vi "Get Default Value.vi"(8 "error in":errorcluster, 9 "project refnum":refnum<vi>, 10 "measurement_signature":T2, 11 "gRPCid in":T1) -> (0 "error out":errorcluster, 3 "default value":variant)   [LabVIEW 2021, in "NI Measurement V2 Client Generator Runtime.lvlib"]
uses:
  NI Measurement V2 Client Generator Runtime.lvlib
  <vilib>/gRPC/Generated APIs/ni/measurementlink/measurement/v2/Measurement Service Client V2/RPC Messages/ni_measurementlink_measurement_v2_MeasurementSignature.ctl
  <vilib>/gRPC/Generated APIs/ni/measurementlink/measurement/v2/Measurement Service Client V2/RPC Messages/ni_measurementlink_measurement_v2_ConfigurationParameter.ctl
  <vilib>/gRPC/Generated APIs/ni/measurementlink/measurement/v2/Measurement Service Client V2/RPC Messages/google_protobuf_Field_Kind.ctl
  <vilib>/gRPC/Generated APIs/ni/measurementlink/measurement/v2/Measurement Service Client V2/RPC Messages/ni_measurementlink_measurement_v2_ConfigurationParameter_AnnotationsEntry.ctl
  <vilib>/gRPC/Generated APIs/ni/measurementlink/measurement/v2/Measurement Service Client V2/RPC Messages/google_protobuf_Any.ctl
  <vilib>/gRPC/Generated APIs/ni/measurementlink/measurement/v2/Measurement Service Client V2/RPC Messages/ni_measurementlink_measurement_v2_Output.ctl
  <vilib>/gRPC/Generated APIs/ni/measurementlink/measurement/v2/Measurement Service Client V2/RPC Messages/ni_measurementlink_measurement_v2_Output_AnnotationsEntry.ctl
  <vilib>/gRPC/LabVIEW gRPC Library/Shared/grpcId.ctl
  <vilib>/Utility/traverseref.llb/TRef TravTarget.ctl
  Client Generator Error Strings Global.vi
  <vilib>/gRPC/LabVIEW gRPC Library/grpc-lvsupport-release.lvlib
  <vilib>/Utility/traverseref.llb/VI Scripting - Traverse.lvlib
  <vilib>/gRPC/Generated APIs/ni/measurementlink/measurement/v2/Measurement Service Client V2/Measurement Service Client V2.lvlib
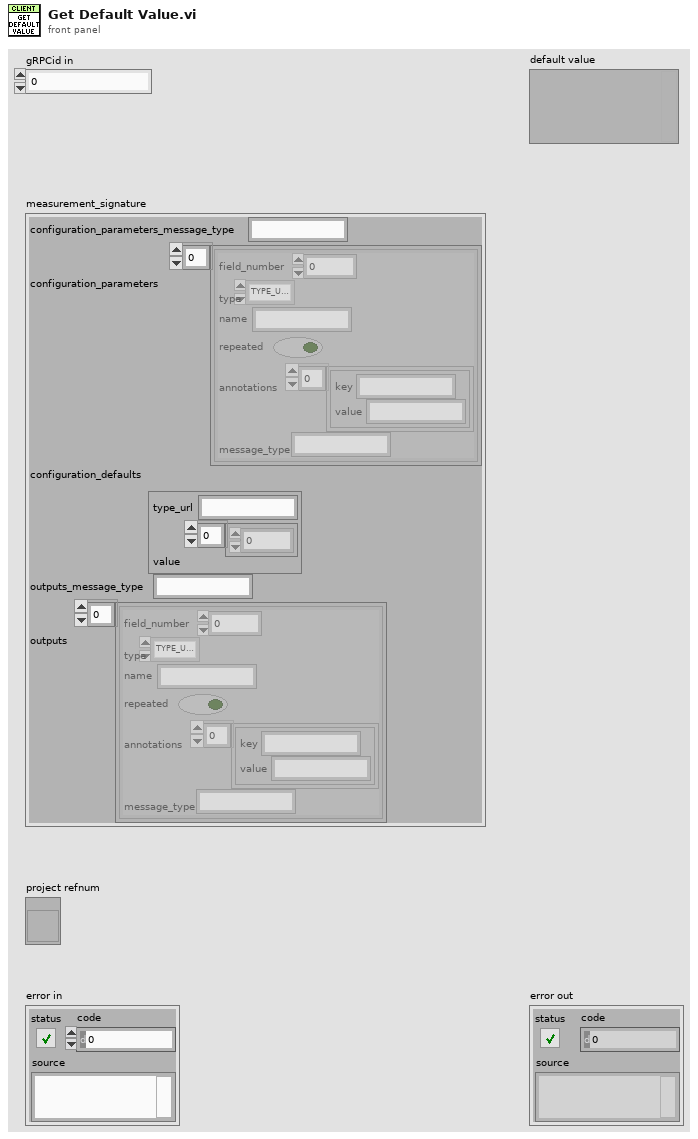
[diagram p1: front panel]
types:
  T1 = typedef "grpc-lvsupport-release.lvlib/grpcId.ctl" = u64
  T2 = typedef "Measurement Service Client V2.lvlib/ni_measurementlink_measurement_v2_MeasurementSignature.ctl" = cluster{"configuration_parameters_message_type":string, "configuration_parameters":T3[], "configuration_defaults":T6, "outputs_message_type":string, "outputs":T7[]}
  T3 = typedef "Measurement Service Client V2.lvlib/ni_measurementlink_measurement_v2_ConfigurationParameter.ctl" = cluster{"field_number":i32, "type":T4, "name":string, "repeated":bool, "annotations":T5[], "message_type":string}
  T4 = typedef "Measurement Service Client V2.lvlib/google_protobuf_Field_Kind.ctl" = enum32{"TYPE_UNKNOWN", "TYPE_DOUBLE", "TYPE_FLOAT", "TYPE_INT64", "TYPE_UINT64", "TYPE_INT32", "TYPE_FIXED64", "TYPE_FIXED32", "TYPE_BOOL", "TYPE_STRING", "TYPE_GROUP", "TYPE_MESSAGE", "TYPE_BYTES", "TYPE_UINT32", "TYPE_ENUM", "TYPE_SFIXED32", "TYPE_SFIXED64", "TYPE_SINT32", "TYPE_SINT64"}
  T5 = typedef "Measurement Service Client V2.lvlib/ni_measurementlink_measurement_v2_ConfigurationParameter_AnnotationsEntry.ctl" = cluster{"key":string, "value":string}
  T6 = typedef "Measurement Service Client V2.lvlib/google_protobuf_Any.ctl" = cluster{"type_url":string, "value":u8[]}
  T7 = typedef "Measurement Service Client V2.lvlib/ni_measurementlink_measurement_v2_Output.ctl" = cluster{"field_number":i32, "type":T4, "name":string, "repeated":bool, "annotations":T8[], "message_type":string}
  T8 = typedef "Measurement Service Client V2.lvlib/ni_measurementlink_measurement_v2_Output_AnnotationsEntry.ctl" = cluster{"key":string, "value":string}
  T9 = typedef "TRef TravTarget.ctl" = enum16{"FP", "BD", "Other"}
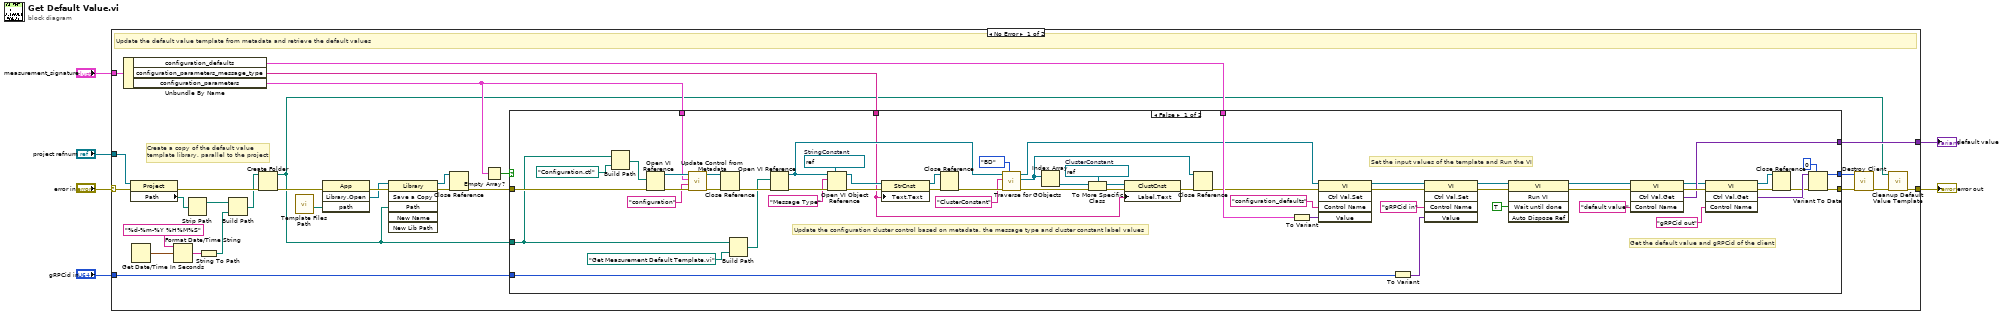
[diagram p0: block diagram]
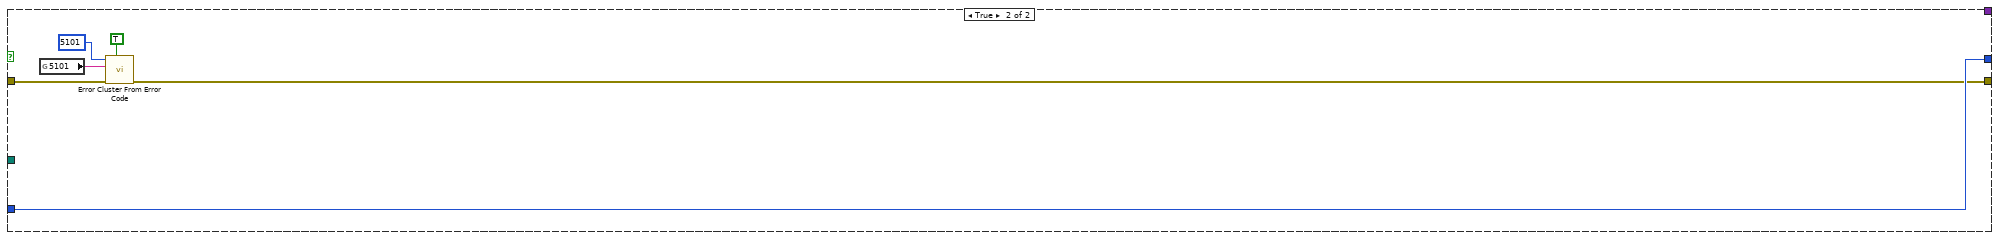
[diagram p2: hidden frame]
diagram:
  n1 = case shown="No Error" "error in" {
    selector: "error in" -> [w35 w101]
    tunnel: [w21 w101] -> w5
    tunnel: "measurement_signature" -> [w15 _]
    tunnel: "gRPCid in" -> [w33 _]
    tunnel: [w32 _] -> w2
    tunnel: "project refnum" -> [w30 _]
    frame No Error {
      # "Create a copy of the default value\ntemplate library, parallel to the project"
      # "Update the default value template from metadata and retrieve the default values"
      n2 = Unbundle By Name(w15) -> ("configuration_defaults"=w34:T6, "configuration_parameters_message_type"=w31:string, "configuration_parameters"=w10:T3[])
      n3 = property class="Project"(reference=w30, error in=w35) -> (error out=w26:errorcluster, "Path"=w29:path)  [unwired: 1 out]
      n4 = Get Date/Time In Seconds() -> (seconds since 1Jan1904=w28:timestamp)
      n5 = Format Date/Time String(time format string (%c)="%d-%m-%Y %H%M%S", seconds (now)=w28) -> (date/time string=w17:string)  [unwired: 1 in]
      n6 = Strip Path(path=w29) -> (stripped path=w27:path)  [unwired: 1 out]
      n7 = String To Path(string=w17) -> (path=w16:path)
      n8 = Build Path(base path=w27, name or relative path=w16) -> (appended path=w24:path)
      n9 = Create Folder(path (use dialog)=w24, error in=w26) -> (created path=w9:path, error out=w25:errorcluster)  [unwired: 1 in, 1 out]
      n10 = call "Template Files Path.vi"() -> ("default template path"=w22:path)  [unwired: 9 in, 2 out]
      n11 = invoke class="App" method="Library.Open"(error in=w25, "path"=w22) -> (error out=w23:errorcluster, "Open Library"=w14:refnum<vi>)  [unwired: 2 in, 2 out]
      n12 = invoke class="Library" method="Save a Copy"(reference=w14, error in=w23, "Path"=w9) -> (reference out=w11:refnum<vi>, error out=w13:errorcluster)  [unwired: 3 in, 4 out]
      n13 = Close Reference(reference=w11, error in (no error)=w13) -> (error out=w12:errorcluster)
      n14 = Empty Array?(array=w10) -> (empty?=w7:bool)
      n15 = case shown="False" w7 {
        tunnel: w34 -> [w83 _]
        tunnel: w33 -> [w79 w100]
        tunnel: [w70 _] -> w32
        tunnel: w31 -> [w54 _]
        tunnel: [w50 w97] -> w19
        tunnel: [w47 w100] -> w18
        tunnel: w12 -> [w46 w95]
        tunnel: w10 -> [w36 _]
        tunnel: w9 -> [w37 _]
        frame False {
          w57 = refnum<vi> refnum  # ClusterConstant
          w90 = refnum<vi> refnum  # StringConstant
          # "Get the default value and gRPCid of the client"
          # "Set the input values of the template and Run the VI"
          # "Update the configuration cluster control based on metadata, the message type and cluster constant label values"
          n16 = Build Path(base path=w37, name or relative path=path "Configuration.ctl") -> (appended path=w40:path)
          n17 = Open VI Reference(vi path=w40, error in (no error)=w46) -> (vi reference=w41:refnum<vi>, error out=w42:errorcluster)  [unwired: 4 in]
          n18 = call "Update Control from Metadata.vi"("error in"=w42, "control name"="configuration", "parameter data"=w36, "vi refnum in"=w41) -> ("error out"=w44:errorcluster, "vi refnum out"=w43:refnum<vi>)  [unwired: 6 in]
          n19 = Close Reference(reference=w43, error in (no error)=w44) -> (error out=w94:errorcluster)
          n20 = Build Path(base path=w37, name or relative path=path "Get Measurement Default Template.vi") -> (appended path=w52:path)
          n21 = Open VI Reference(vi path=w52, error in (no error)=w94) -> (vi reference=w61:refnum<vi>, error out=w93:errorcluster)  [unwired: 4 in]
          n22 = Open VI Object Reference(7:w90, 8:w93, 10:"Message Type" ("name/order"), 11:w61) -> (0:w91:errorcluster, 3:w88:refnum<vi>)
          n23 = property class="StrCnst"(reference=w88, error in=w91, "Text.Text"=w54) -> (reference out=w87:refnum<vi>, error out=w89:errorcluster)
          n24 = Close Reference(reference=w87, error in (no error)=w89) -> (error out=w86:errorcluster)
          n25 = call <vilib>:"Traverse for GObjects.vi"("Traverse Target"=TRef_TravTarget."BD", "error in (no error)"=w86, "Class Name"="ClusterConstant", "VI Refnum"=w61) -> ("error out"=w58:errorcluster, "References"=w51:refnum<vi>[], "dup VI Refnum"=w64:refnum<vi>)  [unwired: 4 in, 1 out]
          n26 = Index Array(array=w51) -> (element=w56:refnum<vi>)  [unwired: 1 in]
          n27 = To More Specific Class(target class=w57, reference=w56, error in=w58) -> (specific class reference=w55:refnum<vi>, error out=w59:errorcluster)
          n28 = property class="ClustCnst"(reference=w55, error in=w59, "Label.Text"=w54) -> (error out=w60:errorcluster)  [unwired: 1 out]
          n29 = Close Reference(reference=w51, error in (no error)=w60) -> (error out=w53:errorcluster)
          n30 = To Variant(anything=w83) -> (Variant=w82:variant)
          n31 = invoke class="VI" method="Ctrl Val.Set"(reference=w64, error in=w53, "Control Name"="configuration_defaults", "Value"=w82) -> (reference out=w80:refnum<vi>, error out=w85:errorcluster)  [unwired: 1 in, 3 out]
          n32 = To Variant(anything=w79) -> (Variant=w78:variant)
          n33 = invoke class="VI" method="Ctrl Val.Set"(reference=w80, error in=w85, "Control Name"="gRPCid in", "Value"=w78) -> (reference out=w75:refnum<vi>, error out=w81:errorcluster)  [unwired: 1 in, 3 out]
          n34 = invoke class="VI" method="Run VI"(reference=w75, error in=w81, "Wait until done"=TRUE ("Wait Until Done")) -> (reference out=w72:refnum<vi>, error out=w76:errorcluster)  [unwired: 2 in, 3 out]
          n35 = invoke class="VI" method="Ctrl Val.Get"(reference=w72, error in=w76, "Control Name"="default value") -> (reference out=w68:refnum<vi>, error out=w73:errorcluster, "Get Control Value Variant"=w70:variant)  [unwired: 1 in, 1 out]
          n36 = invoke class="VI" method="Ctrl Val.Get"(reference=w68, error in=w73, "Control Name"="gRPCid out") -> (reference out=w48:refnum<vi>, error out=w69:errorcluster, "Get Control Value Variant"=w66:variant)  [unwired: 1 in, 1 out]
          n37 = Close Reference(reference=w48, error in (no error)=w69) -> (error out=w49:errorcluster)
          n38 = Variant To Data(error in=w49, type=T1 0 ("gRPCid in"), Variant=w66) -> (data=w47:T1, error out=w50:errorcluster)
        }
        frame True {
          n39 = global read "Client Generator Error Strings Global.vi" "5101"() -> (w99:string)
          n40 = call <vilib>:"Error Cluster From Error Code.vi"("show call chain? (False)"=TRUE, "error in (no error)"=w95, "error message (\"\")"=w99, "error code (0)"=5101) -> ("error out"=w97:errorcluster)  [unwired: 5 in]
        }
      }
      n41 = call <vilib>:"Destroy Client.vi"("error in"=w19, "gRPC ID"=w18) -> ("error out"=w20:errorcluster)  [unwired: 9 in]
      n42 = call "Cleanup Default Value Template.vi"("error in"=w20, "temporary template path"=w9) -> ("error out"=w21:errorcluster)  [unwired: 9 in]
    }
    frame Error {
      # "Pass"
    }
  }
  "error out" <- w5
  "default value" <- w2
